vi "Update Configuration.vi"(8 "error in (no error)":errorcluster, 11 "CIFPlugin in":refnum<class "CAN_Reader_NIXNET_Plugin.lvclass">) -> (0 "error out":errorcluster, 3 "CIFPlugin out":refnum<class "CAN_Reader_NIXNET_Plugin.lvclass">)   [LabVIEW 2021, in "CAN_Reader_NIXNET_Plugin.lvclass"]
uses:
  CAN_Reader_NIXNET_Plugin.lvclass
  C:/Program Files/National Instruments/LabVIEW 2021/vi.lib/CIF Foundation/CIF Core/CIFCore/Class/CIFCorePlugin.lvclass
  CAN_Reader_NIXNET_Plugin.lvclass/CAN_Reader_NIXNET_Plugin.ctl
  <vilib>/CIF Foundation/CIF Core/CIFCore/Class/CIFCorePlugin.lvclass/CIFCorePlugin.ctl
  <vilib>/CIF Foundation/CIF Core/CIFCore/Class/Accessors/Write Configuration Change.vi
  <vilib>/CIF Foundation/CIF Channels Core/ChannelCommon/Utilities/Create FIFO Config.vi
  <vilib>/CIF Foundation/CIF Core/CIFCore/Class/Utilities/Channels/Increase Channel Buffer.vi
  <vilib>/CIF Foundation/CIF Core/CIFCore/Class/CIFCorePlugin.lvclass
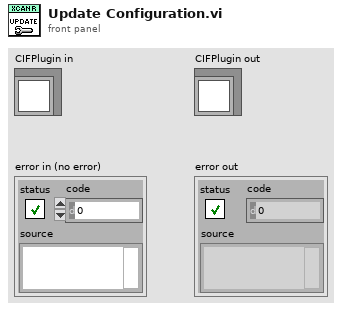
[diagram p1: front panel]
types:
  T1 = typedef "CAN_Reader_NIXNET_Common.lvlib/Configuration.ctl" = cluster{"Common":T2, "RX Interface":string, "Port Configuration":T4, "Timeout (ms)":i32, "Frames to read":i32, "Filter":T7}
  T2 = typedef "CIFCoreCommon.lvlib/Common Plugin Configuration.ctl" = cluster{"Period (s)":dbl, "Offset (us)":i32, "Priority":i32, "Processor":i32, "External Clock":T3}
  T3 = typedef "CIFCoreCommon.lvlib/External Clock Config.ctl" = cluster{"ClockID":u8, "Clock Name":string, "Publish Clock":bool, "Convert Data Timestamps":bool, "Plugin Timing Source":bool}
  T4 = typedef "CAN_RW_CORE.lvclass/CAN Port Configuration.ctl" = cluster{"Mode":T5, "Baud Rate":u64, "Temination On":bool, "Subordinate":bool, "Echo TX":bool, "FD Config":T6}
  T5 = typedef "CAN_RW_CORE.lvclass/CAN Mode.ctl" = enum16{"CAN 2.0", "CAN FD"}
  T6 = typedef "CAN_RW_CORE.lvclass/FD Config.ctl" = cluster{"FD Baud Rate":u64, "ISO Mode":bool, "BRS Enabled":bool}
  T7 = typedef "CAN_RW_CORE.lvclass/CAN Filter.ctl" = cluster{"Allow List (ID)":u32[], "Deny List (ID)":u32[]}
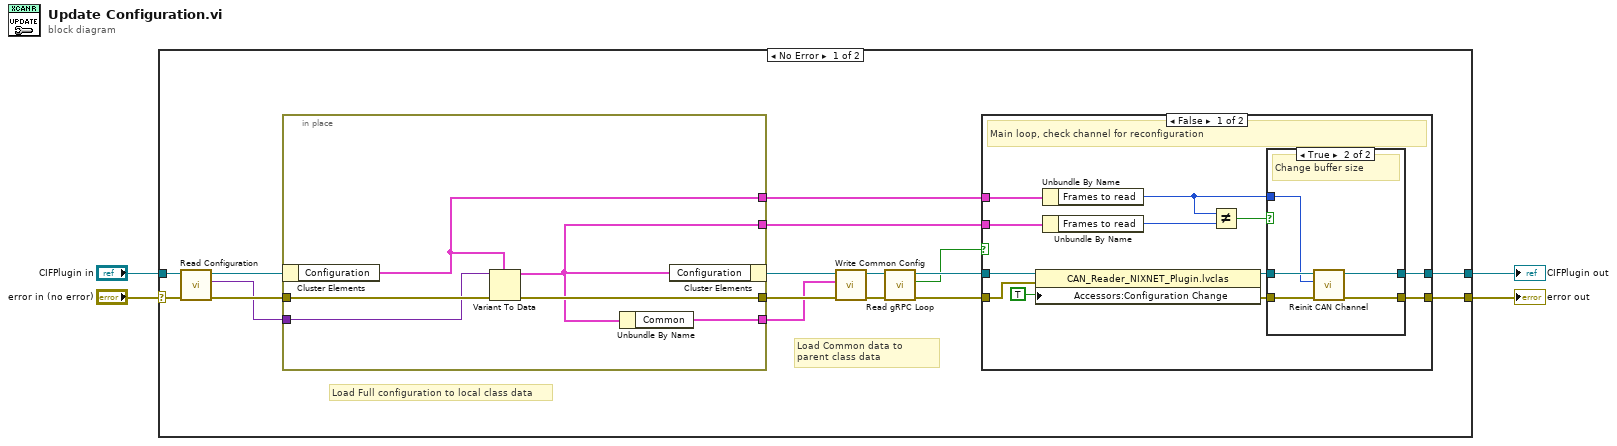
[diagram p0: block diagram]
diagram:
  n1 = case shown="No Error" "error in (no error)" {
    selector: "error in (no error)" -> [w17 w49]
    tunnel: "CIFPlugin in" -> [w18 w50]
    tunnel: [w5 w50] -> w1
    tunnel: [w6 w49] -> w3
    frame No Error {
      # "Load Common data to parent class data"
      # "Load Full configuration to local class data"
      n2 = call <vilib>:"Read Configuration.vi"("error in"=w17, "CIFCorePlugin in"=w18) -> ("error out"=w16:errorcluster, "Configuration Data"=w15:variant, "CIFCorePlugin out"=w14:refnum<class "CAN_Reader_NIXNET_Plugin.lvclass">)  [unwired: 7 in]
      n3 = in-place {
        in-place-border: [w48] -> w21
        in-place-border: w16 -> [w47]
        in-place-border: w15 -> [w46]
        in-place-border: [w45] -> w20
        in-place-border: [w44] -> w8
        in-place-border: [w43] -> w7
        n4 = in-place-cluster #1(w14) -> ("Configuration"=w44:T1)
        n5 = Variant To Data(error in=w47, type=w44, Variant=w46) -> (data=w43:T1, error out=w48:errorcluster)
        n6 = Unbundle By Name(w43) -> ("Common"=w45:T2)
        n7 = in-place-cluster #1("Configuration"=w43) -> (w19:refnum<class "CAN_Reader_NIXNET_Plugin.lvclass">)
      }
      n8 = call <vilib>:"Write Common Config.vi"("error in (no error)"=w21, "Common"=w20, "CIFTemplateNode in"=w19) -> ("error out"=w12:errorcluster, "CIFTemplateNode out"=w13:refnum<class "CAN_Reader_NIXNET_Plugin.lvclass">)  [unwired: 7 in]
      n9 = call <vilib>:"Read gRPC Loop.vi"("error in (no error)"=w12, "CIFCorePlugin in"=w13) -> ("error out"=w10:errorcluster, "gRPC Loop"=w9:bool, "CIFCorePlugin out"=w11:refnum<class "CAN_Reader_NIXNET_Plugin.lvclass">)  [unwired: 7 in]
      n10 = case shown="False" w9 {
        tunnel: w8 -> [w32 _]
        tunnel: w7 -> [w31 _]
        tunnel: [w27 w42] -> w5
        tunnel: [w26 w41] -> w6
        tunnel: w11 -> [w23 w42]
        tunnel: w10 -> [w22 w41]
        frame False {
          # "Main loop, check channel for reconfiguration"
          n11 = property class="CAN_Reader_NIXNET_Plugin.lvclas"(reference=w23, error in=w22, "Accessors:Configuration Change"=TRUE ("Configuration Change")) -> (reference out=w29:refnum<class "CAN_Reader_NIXNET_Plugin.lvclass">, error out=w28:errorcluster)
          n12 = Unbundle By Name(w32) -> ("Frames to read"=w24:i32)
          n13 = Unbundle By Name(w31) -> ("Frames to read"=w30:i32)
          n14 = Not Equal?(x=w24, y=w30) -> (x != y?=w25:bool)
          n15 = case shown="True" w25 {
            tunnel: w29 -> [w35 w40]
            tunnel: w28 -> [w34 w39]
            tunnel: [w35 w37] -> w27
            tunnel: [w34 w38] -> w26
            tunnel: w24 -> [_ w36]
            frame False {
              # "No buffer change"
            }
            frame True {
              # "Change buffer size"
              n16 = call "Reinit CAN Channel.vi"("error in (no error)"=w39, "Configuration.Frames to read"=w36, "CAN_Reader_NIXNET"=w40) -> ("error out"=w38:errorcluster, "CAN_Reader_NIXNET"=w37:refnum<class "CAN_Reader_NIXNET_Plugin.lvclass">)  [unwired: 7 in]
            }
          }
        }
        frame True {
          # "gRPC loop.  Only update the configuration data."
        }
      }
    }
    frame Error {
    }
  }
  "error out" <- w3
  "CIFPlugin out" <- w1
